vi "raspberry_pi_control_panel.vi"() -> ()   [LabVIEW 2026]
uses:
  <userlib>/_OpenG.lib/lvdata/lvdata.llb/openg_variant.lvlib
panel:
  in  "stop":bool
  in  "Path":path=path "/Users/johnnychao/Documents/ENGR4903J/Raspberry_PIs/codems_chil_project"
  in  "Kill on Stop":bool
  in  "Action":T1(ring)
  in  "Run":bool
  out "Output":string
  out "Command Preview":string
  in  "Wait for Convergence":bool
  in  "Auto Plot":bool
  in  "Auto Logs":bool
  in  "Monitor Seconds":dbl
  in  "Iterations":dbl
  in  "Nodes":string
  in  "Scenario":string
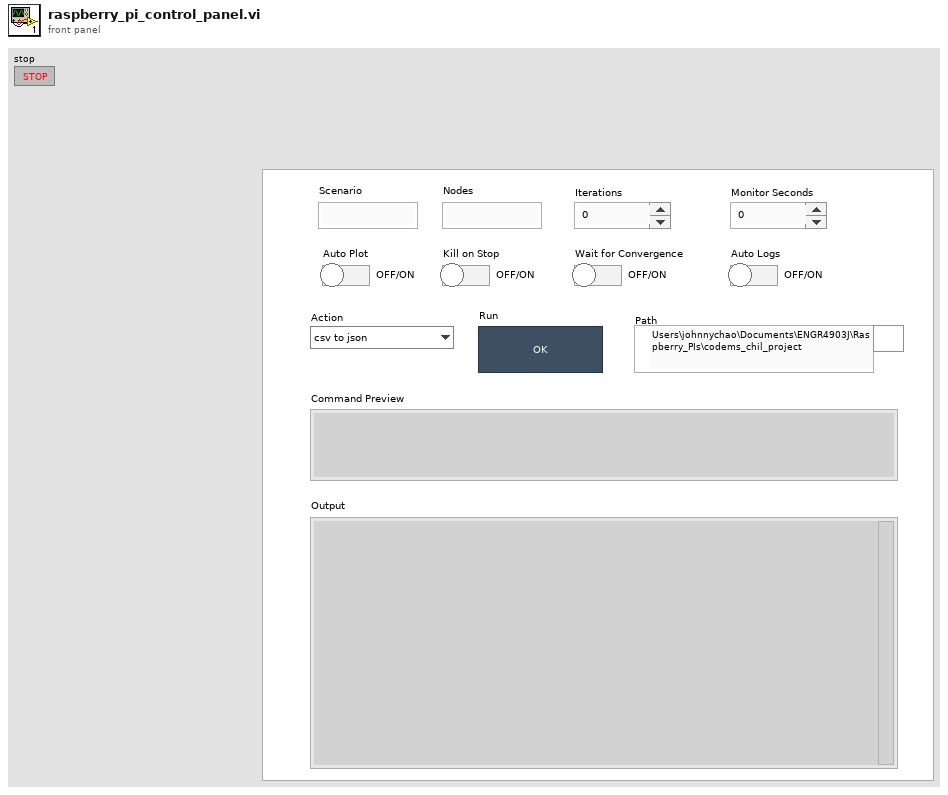
[diagram p1: front panel]
types:
  T1 = enum16{"csv to json", "ping", "deploy", "start", "stop", "monitor", "logs", "centralized-baseline"}
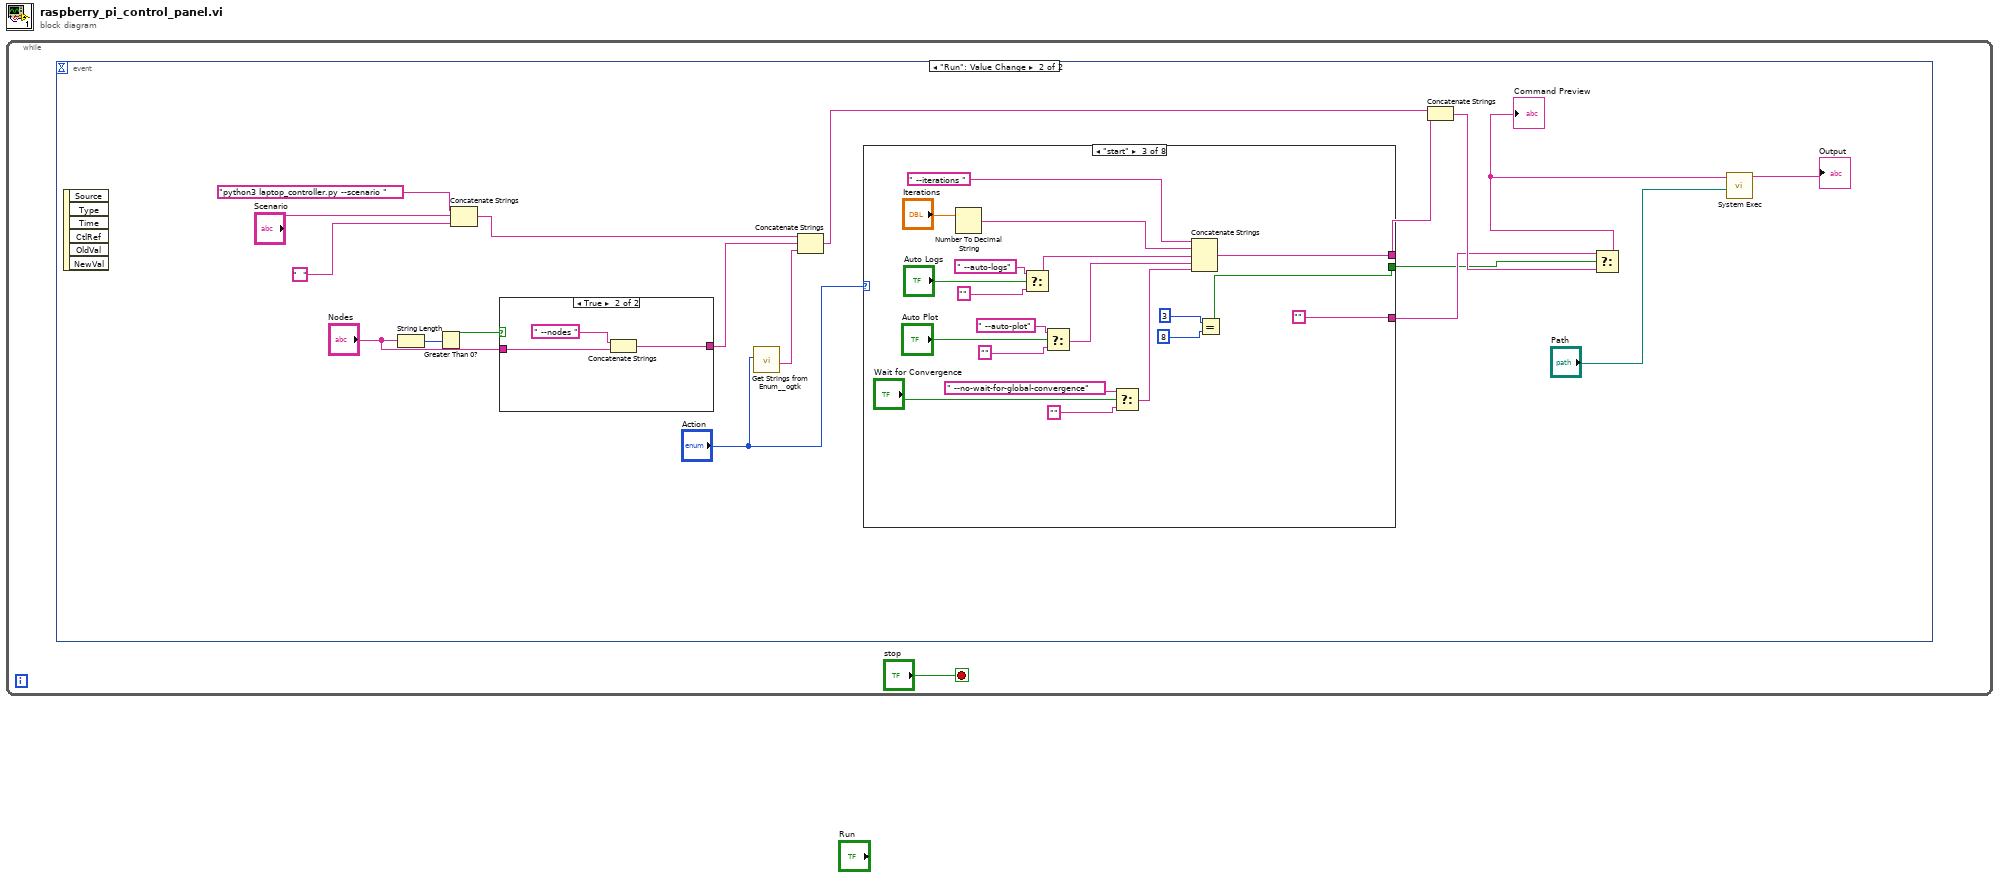
[diagram p0: block diagram]
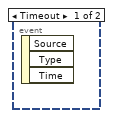
[diagram p2: hidden frame]
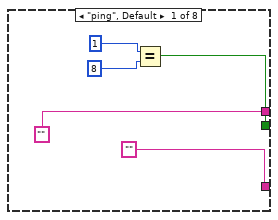
[diagram p3: hidden frame]
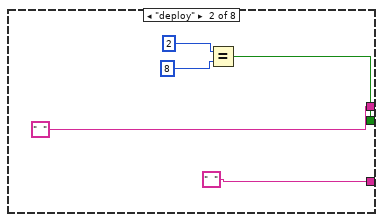
[diagram p4: hidden frame]
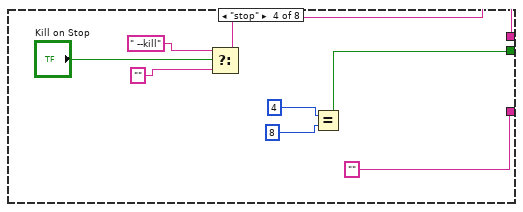
[diagram p5: hidden frame]
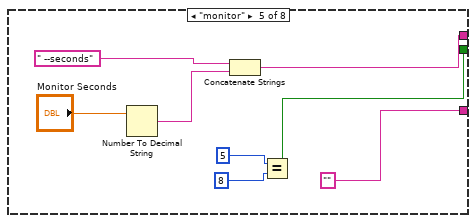
[diagram p6: hidden frame]
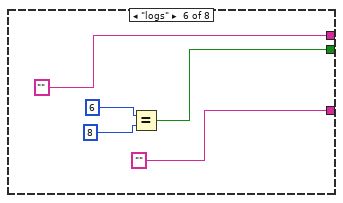
[diagram p7: hidden frame]
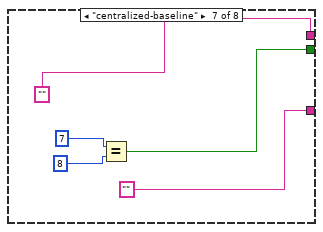
[diagram p8: hidden frame]
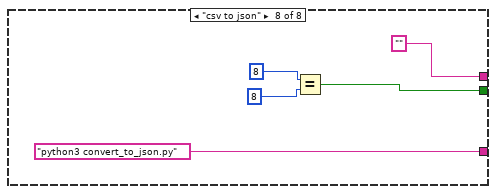
[diagram p9: hidden frame]
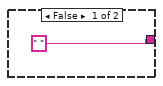
[diagram p10: hidden frame]
diagram:
  n1 = while {
    stop <- "stop" stop-if-true
    n2 = event shown="[1] \"Run\": Value Change" {
      selector: _ -> [_ _]
      dyn-events: _ -> [_ _]
      timeout: _ -> [_ _]
      event Timeout {
        n3 = event-data() -> ()  [unwired: 1 in, 3 out]
      }
      event "Run": Value Change {
        n4 = event-data() -> ()  [unwired: 1 in, 6 out]
        n5 = String Length(string="Nodes") -> (length=w5:i32)
        n6 = Greater Than 0?(x=w5) -> (x > 0?=w6:bool)
        n7 = Concatenate Strings("python3 laptop_controller.py --scenario ", "Scenario", "  ") -> (w7:string)
        n8 = case shown="True" w6 {
          tunnel: [" " w83] -> w9
          tunnel: "Nodes" -> [_ w82]
          frame False {
          }
          frame True {
            n9 = Concatenate Strings(" --nodes ", w82) -> (w83:string)
          }
        }
        n10 = call <userlib>:"Get Strings from Enum__ogtk.vi"("Enum"="Action") -> ("String Value"=w14:string)  [unwired: 7 in, 3 out]
        n11 = Concatenate Strings(w7, w9, w14) -> (w12:string)
        n12 = case shown="\"start\"" "Action" {
          tunnel: ["" "  " w34 w54 w62 "" "" ""] -> w11
          tunnel: [w21 w26 w31 w50 w59 w67 w72 w78] -> w15
          tunnel: ["" "  " "" "" "" "" "" "python3 convert_to_json.py"] -> w16
          frame "ping", Default {
            n13 = Equal?(x=1, y=8) -> (x = y?=w21:bool)
          }
          frame "deploy" {
            n14 = Equal?(x=2, y=8) -> (x = y?=w26:bool)
          }
          frame "start" {
            n15 = Number To Decimal String(number="Iterations") -> (decimal integer string=w38:string)  [unwired: 1 in]
            n16 = Select(t=" --auto-logs", s="Auto Logs", f="") -> (s? t:f=w37:string)
            n17 = Select(t=" --auto-plot", s="Auto Plot", f="") -> (s? t:f=w36:string)
            n18 = Select(t=" --no-wait-for-global-convergence", s="Wait for Convergence", f="") -> (s? t:f=w35:string)
            n19 = Concatenate Strings(" --iterations ", w38, w37, w36, w35) -> (w34:string)
            n20 = Equal?(x=3, y=8) -> (x = y?=w31:bool)
          }
          frame "stop" {
            n21 = Select(t=" --kill", s="Kill on Stop", f="") -> (s? t:f=w54:string)
            n22 = Equal?(x=4, y=8) -> (x = y?=w50:bool)
          }
          frame "monitor" {
            n23 = Number To Decimal String(number="Monitor Seconds") -> (decimal integer string=w63:string)  [unwired: 1 in]
            n24 = Concatenate Strings(" --seconds", w63) -> (w62:string)
            n25 = Equal?(x=5, y=8) -> (x = y?=w59:bool)
          }
          frame "logs" {
            n26 = Equal?(x=6, y=8) -> (x = y?=w67:bool)
          }
          frame "centralized-baseline" {
            n27 = Equal?(x=7, y=8) -> (x = y?=w72:bool)
          }
          frame "csv to json" {
            n28 = Equal?(x=8, y=8) -> (x = y?=w78:bool)
          }
        }
        n29 = Concatenate Strings(w12, w11) -> (w17:string)
        n30 = Select(t=w16, s=w15, f=w17) -> (s? t:f=w18:string)
        "Command Preview" <- w18
        n31 = call <vilib>:"System Exec.vi"("working directory"="Path", "command line"=w18) -> ("standard output"=→"Output":string)  [unwired: 6 in, 3 out]
      }
    }
  }
